vi "Example PWM Measurement.vi"() -> ()   [LabVIEW 2025]
uses:
  wiringPi.lvlib
  Type Defs/GPIO Pins.ctl
  GPIO/Internal/pinMode.Input.vi
  GPIO/Internal/pinMode.Off.vi
  GPIO/Internal/waitForInterrupt.Both.vi
  PWM/Internal/Set PWM.MarkSpace.vi
  PWM/Internal/Set PWM Dutty Cycle.Hardware.vi
  Type Defs/Pull up-down.ctl
panel:
  out "Stoping":bool
  out "Measured Ducy Cycle":dbl format="%#.3g"
  out "Meassured Frec":dbl format="%#.3g"
  in  "Duty Cycle":dbl(knob)=0.5 scale=0.0..1.0 scale format="%.1g"
  in  "PWM Frec":dbl=50.0 format="%#_13g"
  in  "stop":bool
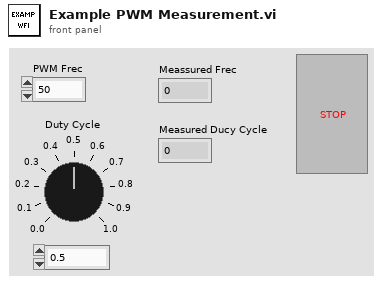
[diagram p1: front panel]
types:
  T1 = typedef "wiringPi.lvlib/Pull up-down.ctl" = enum16{"Off", "Down", "Up"}
  T2 = typedef "wiringPi.lvlib/GPIO Pins.ctl" = enum32{"GPIO0_I2C0_SDA_Pin27", "GPIO1_I2C0_SDA1_Pin28", "GPIO2_I2C1_SDA_Pin3", "GPIO3_I2C1_SCL_Pin5", "GPIO4_GPCLK0_Pin7", "GPIO5_GPCLK1_Pin29", "GPIO6_GPCLK2_Pin31", "GPIO7_SPI_CE1_N_Pin26", "GPIO8_SPI_CE0_N_Pin24", "GPIO9_SPI0_MISO_Pin21", "GPIO10_SPI0_MOSI_Pin19", "GPIO11_SPI0_CLK_Pin23", "GPIO12_PWM0_Pin32", "GPIO13_PWM1_Pin33", "GPIO14_TXD0_Pin8", "GPIO15_RXD0_Pin10", "GPIO16_Pin36", "GPIO17_Pin11", "GPIO18_PWM0_Pin12", "GPIO19_PWM1_Pin35", "GPIO20_GPCLK0_Pin38", "GPIO21_GPCLK1_Pin40", "GPIO22_Pin15", "GPIO23_Pin16", "GPIO24_Pin18", "GPIO25_Pin22", "GPIO26_Pin37", "GPIO27_Pin13"}
  T3 = typedef "wiringPi.lvlib/Edge Mode.ctl" = enum32{"None", "Edge Falling", "Edge Rising", "Both"}
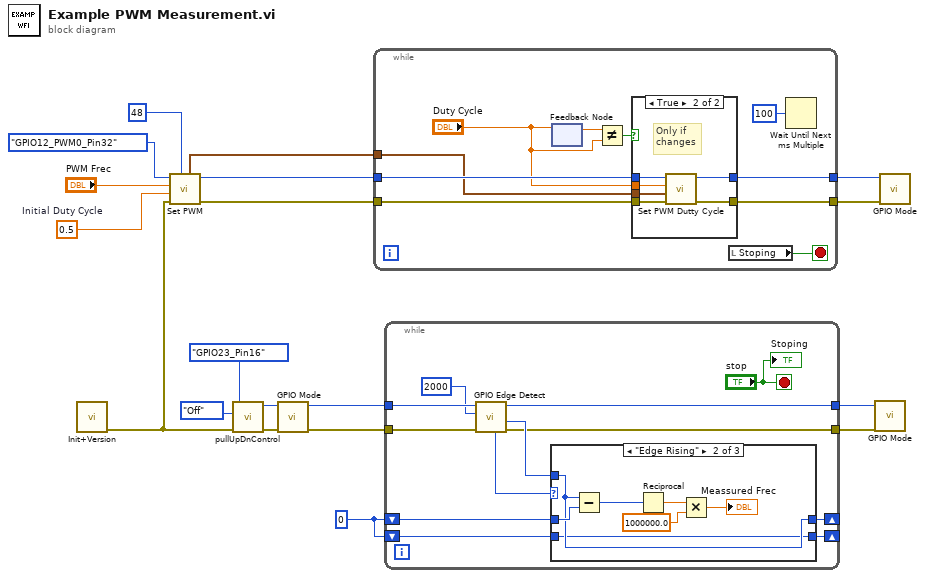
[diagram p0: block diagram]
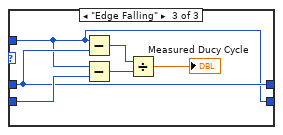
[diagram p4: hidden frame]
diagram:
  w12 = 0.5  # Initial Duty Cycle
  w18 = u64 0 ("TimeStamp (us)")
  n1 = call "Init+Version.vi"() -> ("error out"=w4:errorcluster)  [unwired: 8 in, 3 out]
  n2 = call-poly "Set PWM.vi"("PWM Clock Divider"=48, "error in (no error)"=w4, "Duty Cycle (0-1)"=w12, "PWM Freq (Hz)"="PWM Frec", "RPi PWM Pin in"=GPIO_Pins."GPIO12_PWM0_Pin32" ("RPi Pin")) -> ("error out"=w8:errorcluster, "RPi PWM Pin out"=w13:T2, "PWM Timing"=w9:cluster{"PWM Range":u32, "PWM Data":u32})  [unwired: 2 in, 2 out]
  n3 = call "pullUpDnControl.vi"("error in (no error)"=w4, "Up-Down-Off"=Pull_up-down."Off", "RPi Pin"=GPIO_Pins."GPIO23_Pin16") -> ("error out"=w5:errorcluster, "RPi Pin out"=w3:T2)  [unwired: 7 in]
  n4 = call-poly "GPIO Mode.vi"("error in (no error)"=w5, "RPi Pin"=w3) -> ("error out"=w19:errorcluster, "RPi Pin out"=w15:T2)  [unwired: 8 in]
  n5 = while {
    tunnel: w8 -> [w28]
    tunnel: w13 -> [w26]
    tunnel: w9 -> [w20]
    tunnel: [w25] -> w10
    tunnel: [w24] -> w11
    stop <- w29 stop-if-true
    n6 = feedback-in #1("Duty Cycle") -> ()
    n7 = feedback #1() -> (w23:dbl)  [unwired: 1 in]
    n8 = Not Equal?(x=w23, y="Duty Cycle") -> (x != y?=w22:bool)
    n9 = case shown="True" w22 {
      tunnel: w28 -> [w30 w37]
      tunnel: w26 -> [w31 w36]
      tunnel: [w31 w35] -> w25
      tunnel: [w30 w34] -> w24
      tunnel: "Duty Cycle" -> [_ w33]
      tunnel: w20 -> [_ w32]
      frame False {
      }
      frame True {
        # "Only if\nchanges"
        n10 = call-poly "Set PWM Dutty Cycle.vi"("error in (no error)"=w37, "PWM Timing"=w32, "Duty Cycle (0-1)"=w33, "RPi PWM Pin in"=w36) -> ("error out"=w34:errorcluster, "RPi PWM Pin out"=w35:T2)  [unwired: 6 in]
      }
    }
    n11 = local read "Stoping"() -> (w29:bool)
    n12 = Wait Until Next ms Multiple(millisecond multiple=u32 100) -> ()  [unwired: 1 out]
  }
  n13 = while {
    tunnel: w19 -> [w48]
    tunnel: w15 -> [w49]
    shift-right: [w44] -> _
    shift-left: w18 -> [w41]
    shift-right: [w43] -> _
    shift-left: w18 -> [w42]
    tunnel: [w39] -> w17
    tunnel: [w38] -> w16
    stop <- "stop" stop-if-true
    n14 = call-poly "GPIO Edge Detect.vi"("error in (no error)"=w48, "Timeout (ms)"=2000 ("ms"), "RPi Pin"=w49) -> ("error out"=w39:errorcluster, "TimeStamp (us)"=w46:u64, "RPi Pin out"=w38:T2, "Detected Edge"=w45:T3)  [unwired: 4 in, 1 out]
    n15 = case shown="\"Edge Rising\"" w45 {
      tunnel: w46 -> [_ w53 w61]
      tunnel: [w50 w52 w61] -> w44
      tunnel: [w51 w53 w62] -> w43
      tunnel: w42 -> [w51 w54 w62]
      tunnel: w41 -> [w50 w52 w63]
      frame "None", Default {
      }
      frame "Edge Rising" {
        n16 = Subtract(x=w53, y=w54) -> (x-y=w55:u64)
        n17 = Reciprocal(x=w55) -> (1/x=w58:dbl)
        n18 = Multiply(x=w58, y=1000000.0) -> (x*y=→"Meassured Frec":dbl)
      }
      frame "Edge Falling" {
        n19 = Subtract(x=w61, y=w62) -> (x-y=w60:u64)
        n20 = Subtract(x=w61, y=w63) -> (x-y=w59:u64)
        n21 = Divide(x=w60, y=w59) -> (x/y=→"Measured Ducy Cycle":dbl)
      }
    }
    "Stoping" <- "stop"
  }
  n22 = call-poly "GPIO Mode.vi"("error in (no error)"=w17, "RPi Pin"=w16) -> ()  [unwired: 8 in, 2 out]
  n23 = call-poly "GPIO Mode.vi"("error in (no error)"=w11, "RPi Pin"=w10) -> ()  [unwired: 8 in, 2 out]
